vi "test-traj-generate-14-way.vi"() -> ()   [LabVIEW 2019]
uses:
  <vilib>/Rock Robotics/WPI/ThirdParty/JAS_Junk/TrajLib/Trajectory_Library.lvlib
  <vilib>/Rock Robotics/WPI/ThirdParty/JAS_Junk/TrajLib/TypeDef/TRANSLATION2D.ctl
  <vilib>/Rock Robotics/WPI/ThirdParty/JAS_Junk/TrajLib/TypeDef/ROTATION2D.ctl
  <vilib>/Rock Robotics/WPI/ThirdParty/JAS_Junk/TrajLib/TypeDef/POSE2D.ctl
  <vilib>/Rock Robotics/WPI/ThirdParty/JAS_Junk/TrajLib/TypeDef/TRAJ_CONFIG.ctl
  <vilib>/Analysis/Matrix/Datatypes/RealMatrix.ctl
  <vilib>/Analysis/Matrix/NI_Matrix.lvlib
  <vilib>/Rock Robotics/WPI/ThirdParty/JAS_Junk/TrajLib/TypeDef/POSEwCURVATURE.ctl
  <vilib>/Rock Robotics/WPI/ThirdParty/JAS_Junk/TrajLib/TypeDef/SPLINE_CTRL_VECTOR.ctl
  <vilib>/Rock Robotics/WPI/ThirdParty/JAS_Junk/TrajLib/TypeDef/TRAJECTORY.ctl
  <vilib>/Rock Robotics/WPI/ThirdParty/JAS_Junk/TrajLib/TypeDef/TRAJ_STATE.ctl
  <vilib>/Rock Robotics/WPI/ThirdParty/JAS_Junk/TrajLib/TypeDef/SPLINE.ctl
  <vilib>/Rock Robotics/WPI/ThirdParty/JAS_Junk/TrajLib/TypeDef/DISPLAY_WAYPOINT.ctl
panel:
  in  "Tab Control":T1(tab)
  in  "Interior WAYPOINTS":T2[](array[typedef])=[{"X"=1.848, "Y"=0.765}, {"X"=1.414, "Y"=1.414}, {"X"=0.765, "Y"=1.848}, {"X"=0.0, "Y"=2.0}, {"X"=-0.765, "Y"=1.848}, {"X"=-1.414, "Y"=1.414}, {"X"=-1.848, "Y"=0.765}, {"X"=-2.0, "Y"=0.0}, {"X"=-1.848, "Y"=-0.765}, {"X"=-1.414, "Y"=-1.414}, {"X"=-0.765, "Y"=-1.848}, {"X"=0.0, "Y"=-2.0}, {"X"=0.765, "Y"=-1.848}, {"X"=1.414, "Y"=-1.414}, {"X"=1.848, "Y"=-0.765}] {"Y" format="%14.3f"; "X" format="%14.3f"}
  in  "Initial_Position":T3={"X"=2.0, "Y"=0.0, "ANGLE"=1.571} {"ANGLE" format="%13.3f"; "Y" format="%13.3f"; "X" format="%13.3f"}
  in  "Ending_Position":T3={"X"=2.0, "Y"=0.0, "ANGLE"=1.571} {"ANGLE" format="%13.3f"; "Y" format="%13.3f"; "X" format="%13.3f"}
  out "splines":T4[](array[typedef])
  out "ArrayPoseWithCurvature":T6[](array[typedef]) {"POSE"."ROTATION"."SIN" format="%13.4f"; "POSE"."ROTATION"."COS" format="%13.4f"; "POSE"."ROTATION"."VALUE" format="%13.4f"; "POSE"."TRANSLATION"."Y" format="%14.3f"; "POSE"."TRANSLATION"."X" format="%14.3f"}
  out "PoseCSize":i32
  out "error out 2":errorcluster
  in  "Config":T9={"MaxVelocity"=2.0, "Max Acceleration"=2.0, "StartVelocity"=0.0, "End Velocity"=0.0, "Reversed"=FALSE, "Constraints"=[]} {"End Velocity" format="%20.4f"; "StartVelocity" format="%20.4f"; "Max Acceleration" format="%20.4f"; "MaxVelocity" format="%20.4f"}
  out "initialSpline_Ctrl_Vector":T10
  out "endSpline_Ctrl_Vector":T10
  out "x init":dbl[][](array[numeric])
  out "x final":dbl[][](array[numeric])
  out "y init":dbl[][](array[numeric])
  out "y final":dbl[][](array[numeric])
  out "TRAJECTORY":T11 {"States"."POSE"."ROTATION"."SIN" format="%13.4f"; "States"."POSE"."ROTATION"."COS" format="%13.4f"; "States"."POSE"."ROTATION"."VALUE" format="%13.4f"; "States"."POSE"."TRANSLATION"."Y" format="%14.3f"; "States"."POSE"."TRANSLATION"."X" format="%14.3f"; "TotalTImeSecs" format="%20.3f"}
  out "size(s)":i32
  out "error out":errorcluster
  out "XY Graph":cluster{dbl[], dbl[]}(graph)
  out "Position":cluster{dbl[], dbl[]}(graph)
  out "Done":bool
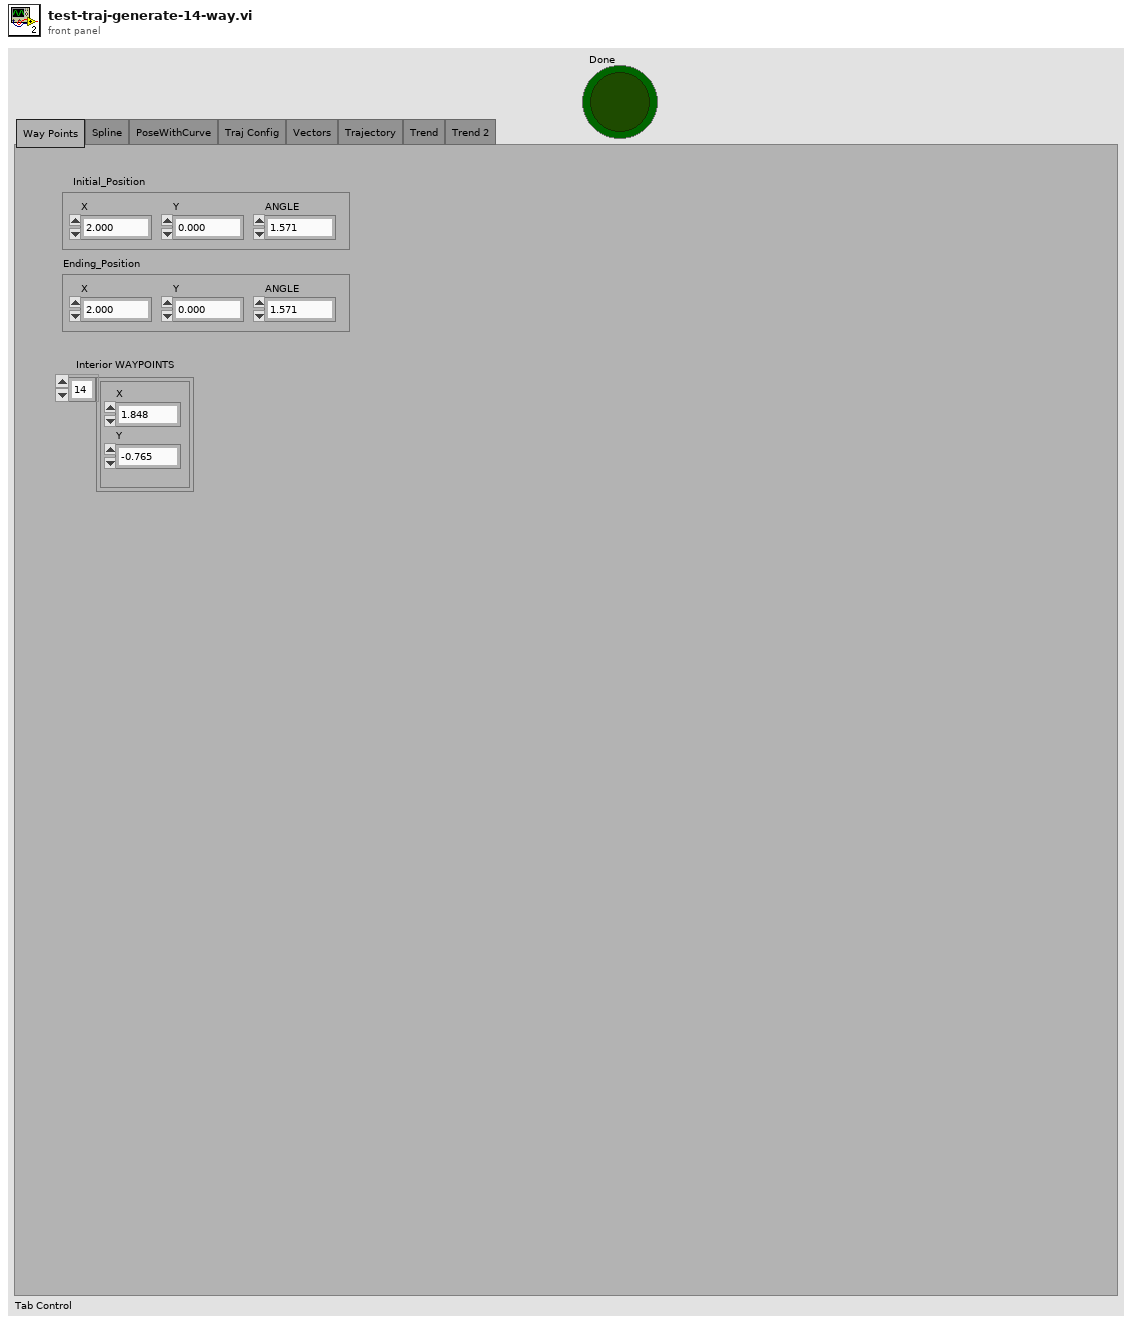
[diagram p1: front panel]
types:
  T1 = enum32{"Way Points", "Spline", "PoseWithCurve", "Traj Config", "Vectors", "Trajectory", "Trend", "Trend 2"}
  T2 = typedef "Trajectory_Library.lvlib/TRANSLATION2D.ctl" = cluster{"X":dbl, "Y":dbl}
  T3 = typedef "Trajectory_Library.lvlib/DISPLAY_WAYPOINT.ctl" = cluster{"X":dbl, "Y":dbl, "ANGLE":dbl}
  T4 = typedef "Trajectory_Library.lvlib/SPLINE.ctl" = cluster{"Degree":i32, "Coefficients":T5}
  T5 = typedef "NI_Matrix.lvlib/RealMatrix.ctl" = dbl[][]
  T6 = typedef "Trajectory_Library.lvlib/POSEwCURVATURE.ctl" = cluster{"CURVATURE":dbl, "POSE":T7}
  T7 = typedef "Trajectory_Library.lvlib/POSE2D.ctl" = cluster{"TRANSLATION":T2, "ROTATION":T8}
  T8 = typedef "Trajectory_Library.lvlib/ROTATION2D.ctl" = cluster{"VALUE":dbl, "COS":dbl, "SIN":dbl}
  T9 = typedef "Trajectory_Library.lvlib/TRAJ_CONFIG.ctl" = cluster{"MaxVelocity":dbl, "Max Acceleration":dbl, "StartVelocity":dbl, "End Velocity":dbl, "Reversed":bool, "Constraints":variant[]}
  T10 = typedef "Trajectory_Library.lvlib/SPLINE_CTRL_VECTOR.ctl" = cluster{"Xs":dbl[], "Ys":dbl[]}
  T11 = typedef "Trajectory_Library.lvlib/TRAJECTORY.ctl" = cluster{"TotalTImeSecs":dbl, "States":T12[]}
  T12 = typedef "Trajectory_Library.lvlib/TRAJ_STATE.ctl" = cluster{"TimeSeconds":dbl, "Velocity":dbl, "Acceleration":dbl, "POSE":T7, "Curvature":dbl}
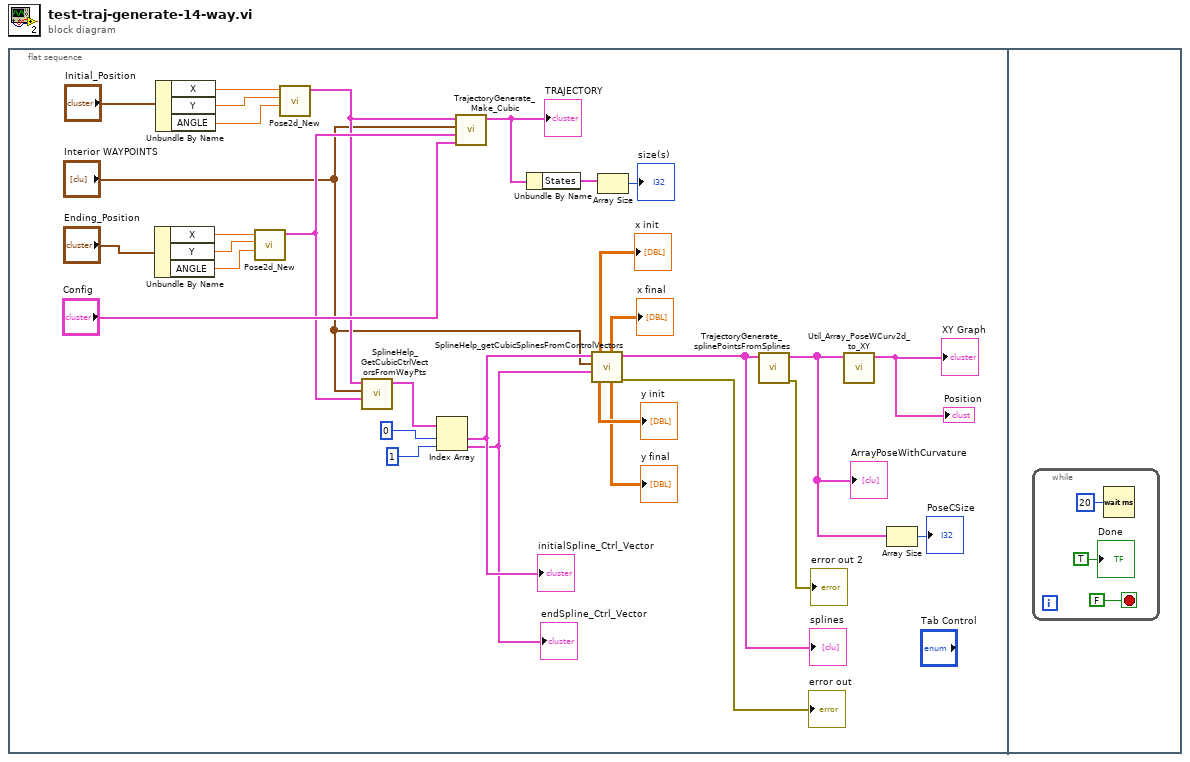
[diagram p0: block diagram]
diagram:
  n1 = flat-sequence {
    frame #0 {
      n2 = Unbundle By Name("Ending_Position") -> ("X"=w25:dbl, "Y"=w24:dbl, "ANGLE"=w23:dbl)
      n3 = Unbundle By Name("Initial_Position") -> ("X"=w28:dbl, "Y"=w27:dbl, "ANGLE"=w26:dbl)
      n4 = call <vilib>:"Pose2d_New.vi"("Heading"=w23, "Y"=w24, "X"=w25) -> ("out POSe"=w21:T7)  [unwired: 8 in]
      n5 = call <vilib>:"Pose2d_New.vi"("Heading"=w26, "Y"=w27, "X"=w28) -> ("out POSe"=w20:T7)  [unwired: 8 in]
      n6 = call <vilib>:"SplineHelp_GetCubicCtrlVectorsFromWayPts.vi"("Enging POSE"=w21, "Interior WAYPOINTS"="Interior WAYPOINTS", "Starting POSE"=w20) -> ("SplineControlVectors"=w8:T10[])  [unwired: 8 in]
      n7 = Index Array(array=w8, index #1=0 ("index"), index #2=1 ("index")) -> (element #1=w7:T10, element #2=w6:T10)
      "initialSpline_Ctrl_Vector" <- w7
      "endSpline_Ctrl_Vector" <- w6
      n8 = call <vilib>:"TrajectoryGenerate_Make_Cubic.vi"("traj_config"="Config", "Enging POSE"=w21, "Interior WAYPOINTS"="Interior WAYPOINTS", "Starting POSE"=w20) -> ("TRAJECTORY"=w16:T11)  [unwired: 6 in, 1 out]
      "TRAJECTORY" <- w16
      n9 = Unbundle By Name(w16) -> ("States"=w15:T12[])
      n10 = call <vilib>:"SplineHelp_getCubicSplinesFromControlVectors.vi"("endCtrlVector"=w6, "InternalWaypoints"="Interior WAYPOINTS", "startCtrlVector"=w7) -> ("error out"=→"error out":errorcluster, "splines"=w18:T4[], "y final"=→"y final":dbl[][], "x final"=→"x final":dbl[][], "y init"=→"y init":dbl[][], "x init"=→"x init":dbl[][])  [unwired: 3 in]
      "splines" <- w18
      n11 = Array Size(array=w15) -> (size(s)=→"size(s)":i32)
      n12 = call <vilib>:"TrajectoryGenerate_splinePointsFromSplines.vi"("inputSPLINE"=w18) -> ("error out"=→"error out 2":errorcluster, "ArrayPoseWithCurvature"=w12:T6[])  [unwired: 9 in]
      "ArrayPoseWithCurvature" <- w12
      n13 = call <vilib>:"Util_Array_PoseWCurv2d_to_XY.vi"("inArrayPoseWCurve"=w12) -> ("outArrayXY"=→"XY Graph" →"Position":cluster{dbl[], dbl[]})  [unwired: 10 in]
      n14 = Array Size(array=w12) -> (size(s)=→"PoseCSize":i32)
    }
    frame #1 {
      n15 = while {
        stop <- FALSE stop-if-true
        n16 = Wait (ms)(milliseconds to wait=u32 20) -> ()  [unwired: 1 out]
        "Done" <- TRUE ("Done")
      }
    }
  }
